vi "Analog Test Bench.vi"() -> ()   [LabVIEW 2021]
uses:
  DAQNavi_AO.lvclass/DAQNavi_AO.lvclass
  DAQNavi_AI.lvclass/DAQNavi_AI.lvclass
  DAQNavi_AI.lvclass/DAQNavi_AI.lvclass/DAQNavi_AI.ctl
  DAQNavi_AO.lvclass/DAQNavi_AO.lvclass/DAQNavi_AO.ctl
panel:
  out "Data In":dbl format="%0.2f"
  in  "stop":bool
  in  "Data out":dbl
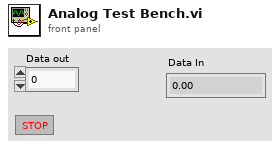
[diagram p1: front panel]
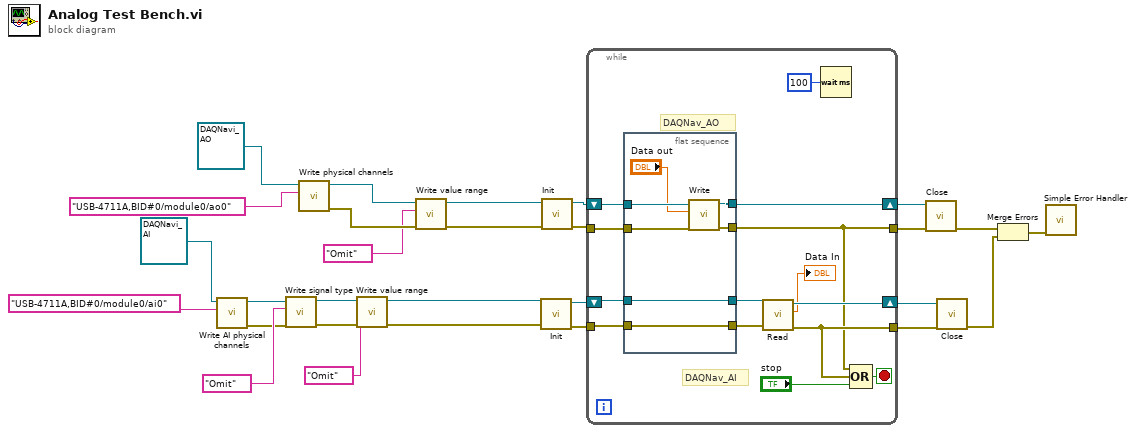
[diagram p0: block diagram]
diagram:
  n1 = call "Write AI physical channels.vi"("physical channels"="USB-4711A,BID#0/module0/ai0", "DAQNavi_AI in"=refnum<class "DAQNavi_AI.lvclass"> refnum) -> ("error out"=w11:errorcluster, "DAQNavi_AI out"=w13:refnum<class "DAQNavi_AI.lvclass">)  [unwired: 8 in]
  n2 = call "Write signal type.vi"("error in (no error)"=w11, "signal type"="Omit", "DAQNavi_AI in"=w13) -> ("error out"=w10:errorcluster, "DAQNavi_AI out"=w9:refnum<class "DAQNavi_AI.lvclass">)  [unwired: 7 in]
  n3 = call "Write physical channels.vi"("physical channels"="USB-4711A,BID#0/module0/ao0", "DAQNavi_AO in"=refnum<class "DAQNavi_AO.lvclass"> refnum) -> ("error out"=w27:errorcluster, "DAQNavi_AO out"=w28:refnum<class "DAQNavi_AO.lvclass">)  [unwired: 8 in]
  n4 = call "Write value range.vi"("error in (no error)"=w10, "value range"="Omit", "DAQNavi_AI in"=w9) -> ("error out"=w7:errorcluster, "DAQNavi_AI out"=w6:refnum<class "DAQNavi_AI.lvclass">)  [unwired: 7 in]
  n5 = call "Write value range.vi"("error in (no error)"=w27, "value range"="Omit", "DAQNavi_AO in"=w28) -> ("error out"=w24:errorcluster, "DAQNavi_AO out"=w25:refnum<class "DAQNavi_AO.lvclass">)  [unwired: 7 in]
  n6 = call-dynamic "Init.vi"("error in (no error)"=w7, "DAQNavi_AI in"=w6) -> ("error out"=w16:errorcluster, "DAQNavi_AI out"=w17:refnum<class "DAQNavi_AI.lvclass">)  [unwired: 8 in]
  n7 = call-dynamic "Init.vi"("error in (no error)"=w24, "DAQNavi_AO in"=w25) -> ("error out"=w23:errorcluster, "DAQNavi_AO out"=w22:refnum<class "DAQNavi_AO.lvclass">)  [unwired: 8 in]
  n8 = while {
    shift-right: [w40] -> w21
    shift-left: w22 -> [w41]
    tunnel: w23 -> [w42]
    tunnel: [w29] -> w20
    tunnel: w16 -> [w34]
    tunnel: [w30] -> w5
    shift-right: [w38] -> w4
    shift-left: w17 -> [w36]
    stop <- w31 stop-if-true
    # "DAQNav_AI"
    # "DAQNav_AO"
    n9 = flat-sequence {
      tunnel: w42 -> [w49]
      tunnel: w41 -> [w48]
      tunnel: [w46] -> w40
      tunnel: [w45] -> w29
      tunnel: [w44] -> w37
      tunnel: w36 -> [w44]
      tunnel: [w43] -> w35
      tunnel: w34 -> [w43]
      frame #0 {
        n10 = call-dynamic "Write.vi"("error in (no error)"=w49, "data in"="Data out", "DAQNavi_AO in"=w48) -> ("error out"=w45:errorcluster, "DAQNavi_AO out"=w46:refnum<class "DAQNavi_AO.lvclass">)  [unwired: 7 in]
      }
    }
    n11 = call-dynamic "Read.vi"("error in (no error)"=w35, "DAQNavi_AI in"=w37) -> ("error out"=w30:errorcluster, "Data Out"=→"Data In":dbl, "DAQNavi_AI out"=w38:refnum<class "DAQNavi_AI.lvclass">)  [unwired: 7 in]
    n12 = Wait (ms)(milliseconds to wait=u32 100) -> ()  [unwired: 1 out]
    n13 = Compound Arithmetic op=OR(w29, w30, "stop") -> (w31:bool)
  }
  n14 = call-dynamic "Close.vi"("error in (no error)"=w20, "DAQNavi_AO in"=w21) -> ("error out"=w3:errorcluster)  [unwired: 8 in, 1 out]
  n15 = call-dynamic "Close.vi"("error in (no error)"=w5, "DAQNavi_AI in"=w4) -> ("error out"=w1:errorcluster)  [unwired: 8 in, 1 out]
  n16 = Merge Errors(w3, w1) -> (w2:errorcluster)
  n17 = call <vilib>:"Simple Error Handler.vi"("error in (no error)"=w2) -> ()  [unwired: 4 in, 5 out]
